vi "SC Deploy Command.vi"(6 "deploying?":bool=TRUE, 7 "close project first?":bool, 8 "error in (no error)":errorcluster, 9 "arguments":string[](array[string]), 10 "title":string, 11 "OK message":string="Done.") -> (0 "error out":errorcluster, 1 "result":string)   [LabVIEW 2023]
doc: "Runs a systemcore-deploy deploy, redeploy or fetch command. When the robot runs a version the project doesn't have (DIVERGED), shows SC Choose Version and runs it again with --resolve; when only the robot has changes (BEHIND), takes them without asking; when the robot's SSH host key changed, asks and runs it again with --trust-new-hostkey. Before a choice that changes the project's files (robot, merge), or before running at all when close project first? is set (a command that always changes them, like checkout), it closes the project, and after showing the result it opens it again."
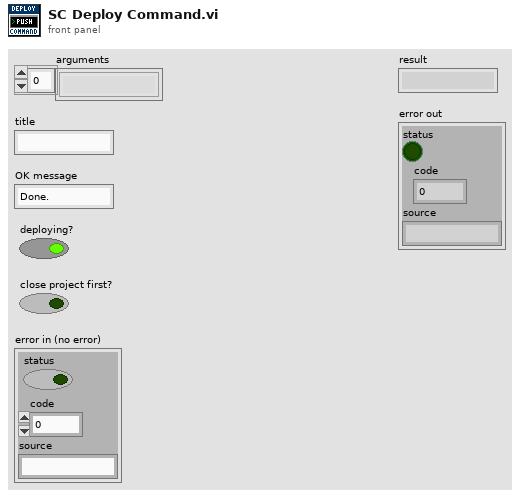
[diagram p1: front panel]
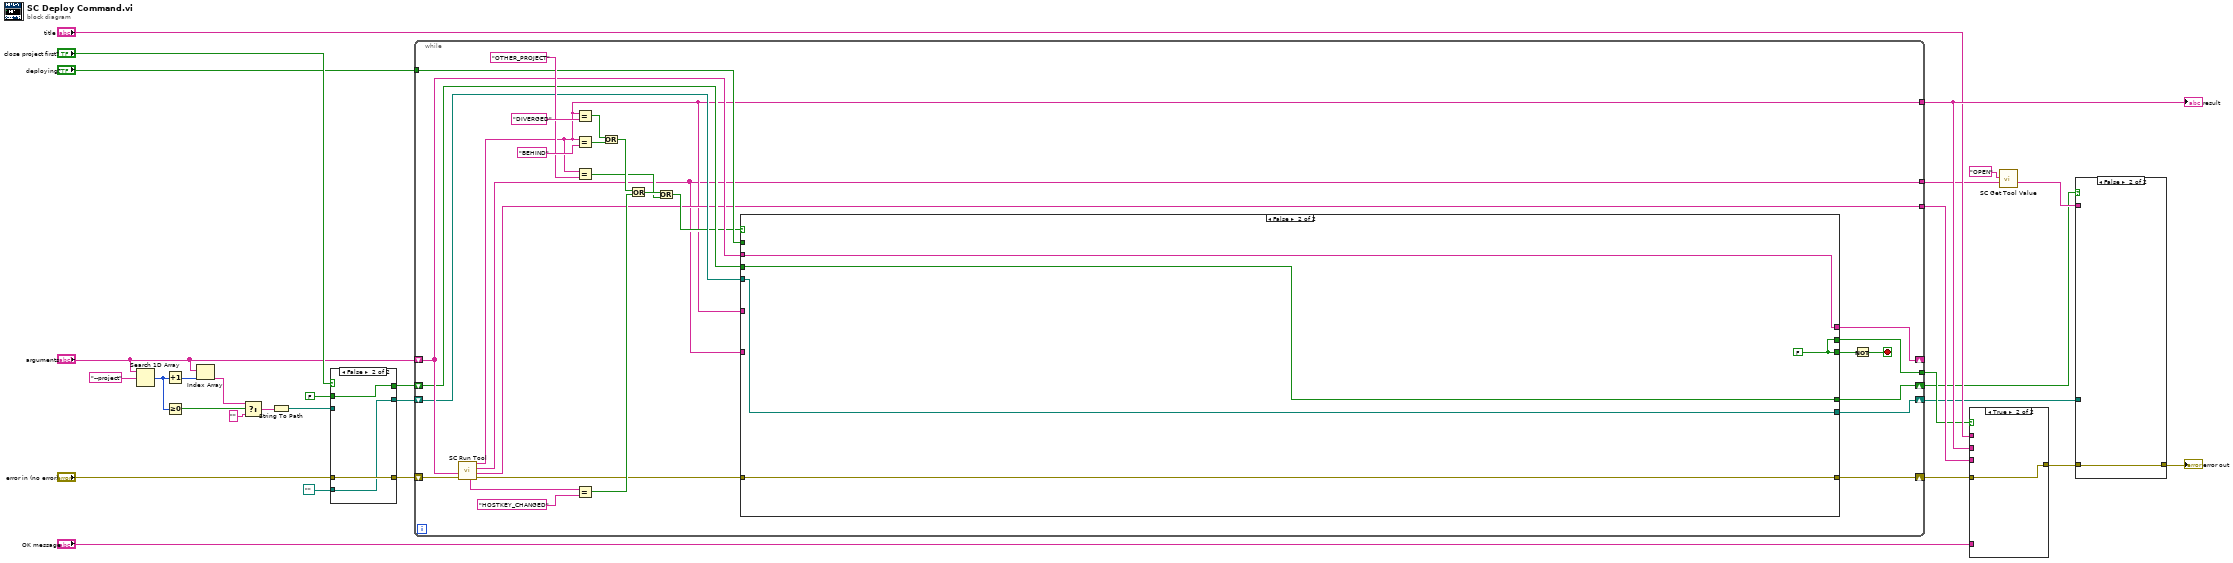
[diagram p0: block diagram]
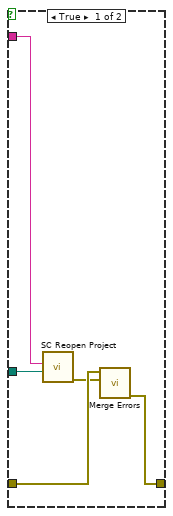
[diagram p2: hidden frame]
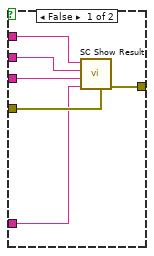
[diagram p3: hidden frame]
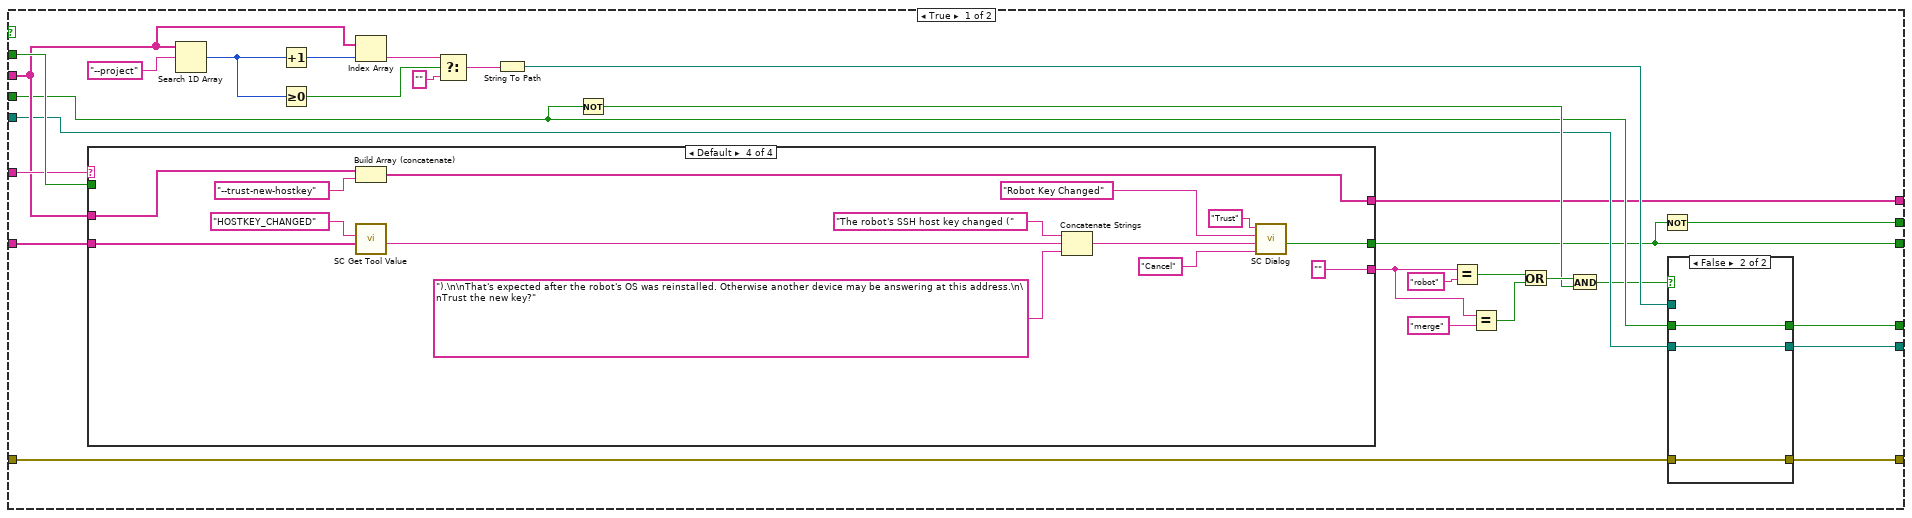
[diagram p4: hidden frame]
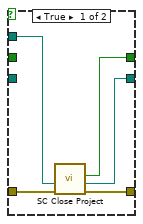
[diagram p5: hidden frame]
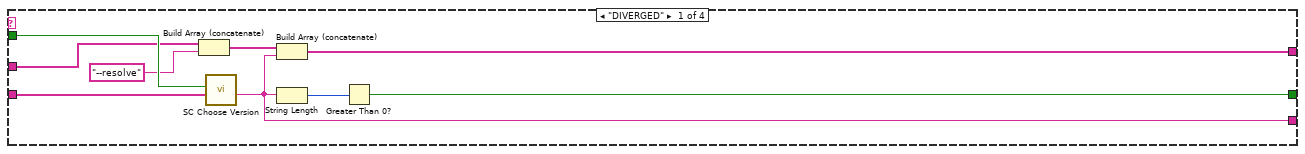
[diagram p6: hidden frame]
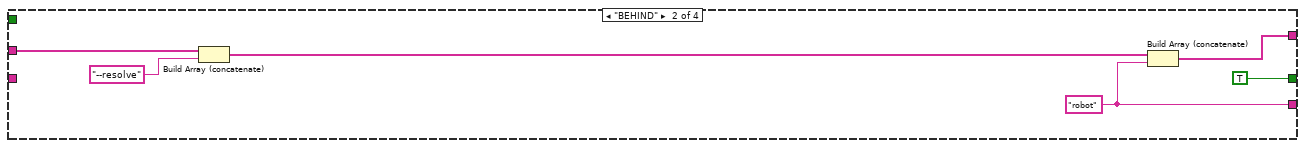
[diagram p7: hidden frame]
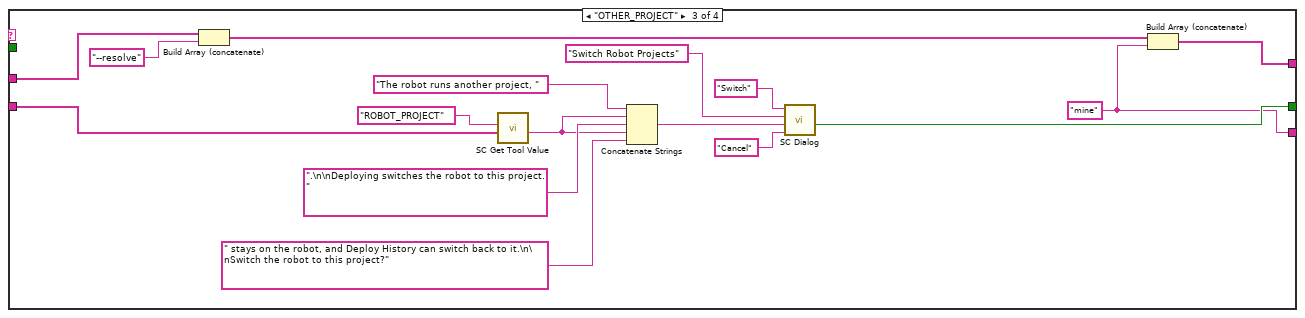
[diagram p8: hidden frame]
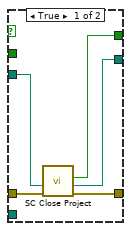
[diagram p9: hidden frame]
diagram:
  n1 = Search 1D Array(1D array="arguments", element="--project") -> (index of element=w28:i32)  [unwired: 1 in]
  n2 = Increment(x=w28) -> (x+1=w29:i32)
  n3 = Greater Or Equal To 0?(x=w28) -> (x >= 0?=w27:bool)
  n4 = Index Array(array="arguments", index=w29) -> (element=w26:string)
  n5 = Select(t=w26, s=w27, f="") -> (s? t:f=w24:string)
  n6 = String To Path(string=w24) -> (path=w20:path)
  n7 = case shown="False" "close project first?" {
    tunnel: "error in (no error)" -> [w35 w38]
    tunnel: FALSE -> [_ w37]
    tunnel: path "" -> [_ w36]
    tunnel: w20 -> [w34 _]
    tunnel: [w33 w38] -> w17
    tunnel: [w32 w37] -> w16
    tunnel: [w31 w36] -> w15
    frame True {
      n8 = call "SC Close Project.vi"("error in (no error)"=w35, "project folder"=w34) -> ("error out"=w33:errorcluster, "project path"=w31:path, "closed?"=w32:bool)  [unwired: 7 in]
    }
    frame False {
    }
  }
  n9 = while {
    shift-right: [w49] -> _
    shift-left: "arguments" -> [w54]
    shift-right: [w48] -> w9
    shift-left: w17 -> [w66]
    shift-right: [w47] -> w1
    shift-left: w16 -> [w51]
    shift-right: [w46] -> w5
    shift-left: w15 -> [w50]
    tunnel: "deploying?" -> [w53]
    tunnel: [w42] -> w13
    tunnel: [w41] -> w12
    tunnel: [w40] -> w8
    tunnel: [w39] -> w7
    stop <- w43 stop-if-true
    n10 = call "SC Run Tool.vi"("error in (no error)"=w66, "arguments"=w54) -> ("error out"=w52:errorcluster, "output"=w42:string, "tool lines"=w39:string[], "result"=w41:string, "result detail"=w63:string)  [unwired: 4 in, 1 out]
    n11 = Equal?(x=w41, y="DIVERGED") -> (x = y?=w61:bool)
    n12 = Equal?(x=w41, y="BEHIND") -> (x = y?=w60:bool)
    n13 = Equal?(x=w41, y="OTHER_PROJECT") -> (x = y?=w55:bool)
    n14 = Equal?(x=w63, y="HOSTKEY_CHANGED") -> (x = y?=w58:bool)
    n15 = Or(x=w61, y=w60) -> (x .or. y?=w59:bool)
    n16 = Or(x=w59, y=w58) -> (x .or. y?=w56:bool)
    n17 = Or(x=w56, y=w55) -> (x .or. y?=w45:bool)
    n18 = case shown="False" w45 {
      tunnel: w54 -> [w84 w153]
      tunnel: w39 -> [w95 _]
      tunnel: w41 -> [w93 _]
      tunnel: w53 -> [w94 _]
      tunnel: w52 -> [w77 w151]
      tunnel: w51 -> [w76 w150]
      tunnel: w50 -> [w75 w149]
      tunnel: [w72 w153] -> w49
      tunnel: [w71 w152] -> w44
      tunnel: [w70 w152] -> w40
      tunnel: [w69 w151] -> w48
      tunnel: [w68 w150] -> w47
      tunnel: [w67 w149] -> w46
      frame True {
        n19 = case shown="Default" w93 {
          tunnel: w84 -> [w109 w118 w124 w139]
          tunnel: w95 -> [w112 _ w134 w148]
          tunnel: w94 -> [w111 _ _ _]
          tunnel: [w106 w115 w121 w137] -> w72
          tunnel: [w105 TRUE w120 w136] -> w71
          tunnel: [w104 w113 w119 ""] -> w91
          frame "DIVERGED" {
            n20 = Build Array (concatenate)(w109, "--resolve") -> (w107:string[])
            n21 = call "SC Choose Version.vi"("tool lines"=w112, "deploying?"=w111) -> ("choice"=w104:string)  [unwired: 9 in]
            n22 = Build Array (concatenate)(w107, w104) -> (w106:string[])
            n23 = String Length(string=w104) -> (length=w110:i32)
            n24 = Greater Than 0?(x=w110) -> (x > 0?=w105:bool)
          }
          frame "BEHIND" {
            w113 = "robot"
            n25 = Build Array (concatenate)(w118, "--resolve") -> (w116:string[])
            n26 = Build Array (concatenate)(w116, w113) -> (w115:string[])
          }
          frame "OTHER_PROJECT" {
            w119 = "mine"
            n27 = Build Array (concatenate)(w124, "--resolve") -> (w122:string[])
            n28 = call "SC Get Tool Value.vi"("tool lines"=w134, "key"="ROBOT_PROJECT") -> ("value"=w130:string)  [unwired: 8 in, 1 out]
            n29 = Concatenate Strings("The robot runs another project, ", w130, ".\n\nDeploying switches the robot to this project. ", w130, " stays on the robot, and Deploy History can switch back to it.\n\nSwitch the robot to this project?") -> (w128:string)
            n30 = call "SC Dialog.vi"("Cancel text"="Cancel", "message"=w128, "window title"="Switch Robot Projects", "OK text"="Switch") -> ("OK?"=w120:bool)  [unwired: 7 in]
            n31 = Build Array (concatenate)(w122, w119) -> (w121:string[])
          }
          frame Default {
            n32 = Build Array (concatenate)(w139, "--trust-new-hostkey") -> (w137:string[])
            n33 = call "SC Get Tool Value.vi"("tool lines"=w148, "key"="HOSTKEY_CHANGED") -> ("value"=w145:string)  [unwired: 8 in, 1 out]
            n34 = Concatenate Strings("The robot's SSH host key changed (", w145, ").\n\nThat's expected after the robot's OS was reinstalled. Otherwise another device may be answering at this address.\n\nTrust the new key?") -> (w143:string)
            n35 = call "SC Dialog.vi"("Cancel text"="Cancel", "message"=w143, "window title"="Robot Key Changed", "OK text"="Trust") -> ("OK?"=w136:bool)  [unwired: 7 in]
          }
        }
        n36 = Search 1D Array(1D array=w84, element="--project") -> (index of element=w82:i32)  [unwired: 1 in]
        n37 = Increment(x=w82) -> (x+1=w83:i32)
        n38 = Greater Or Equal To 0?(x=w82) -> (x >= 0?=w81:bool)
        n39 = Index Array(array=w84, index=w83) -> (element=w80:string)
        n40 = Select(t=w80, s=w81, f="") -> (s? t:f=w78:string)
        n41 = String To Path(string=w78) -> (path=w74:path)
        n42 = Not(x=w76) -> (.not. x?=w86:bool)
        n43 = Equal?(x=w91, y="robot") -> (x = y?=w89:bool)
        n44 = Equal?(x=w91, y="merge") -> (x = y?=w88:bool)
        n45 = Or(x=w89, y=w88) -> (x .or. y?=w87:bool)
        n46 = And(x=w87, y=w86) -> (x .and. y?=w73:bool)
        n47 = Not(x=w71) -> (.not. x?=w70:bool)
        n48 = case shown="False" w73 {
          tunnel: w77 -> [w100 w103]
          tunnel: w76 -> [_ w102]
          tunnel: w75 -> [_ w101]
          tunnel: w74 -> [w99 _]
          tunnel: [w98 w103] -> w69
          tunnel: [w97 w102] -> w68
          tunnel: [w96 w101] -> w67
          frame True {
            n49 = call "SC Close Project.vi"("error in (no error)"=w100, "project folder"=w99) -> ("error out"=w98:errorcluster, "project path"=w96:path, "closed?"=w97:bool)  [unwired: 7 in]
          }
          frame False {
          }
        }
      }
      frame False {
        w152 = FALSE
      }
    }
    n50 = Not(x=w44) -> (.not. x?=w43:bool)
  }
  "result" <- w12
  n51 = case shown="True" w8 {
    tunnel: w13 -> [w158 _]
    tunnel: w12 -> [w157 _]
    tunnel: "title" -> [w156 _]
    tunnel: "OK message" -> [w155 _]
    tunnel: w9 -> [w159 w160]
    tunnel: [w154 w160] -> w3
    frame False {
      n52 = call "SC Show Result.vi"("error in (no error)"=w159, "OK message"=w155, "output"=w158, "result"=w157, "title"=w156) -> ("error out"=w154:errorcluster)  [unwired: 6 in]
    }
    frame True {
    }
  }
  n53 = call "SC Get Tool Value.vi"("tool lines"=w7, "key"="OPEN") -> ("value"=w4:string)  [unwired: 8 in, 1 out]
  n54 = case shown="False" w1 {
    tunnel: w5 -> [w165 _]
    tunnel: w4 -> [w164 _]
    tunnel: w3 -> [w163 w166]
    tunnel: [w161 w166] -> w2
    frame True {
      n55 = call "SC Reopen Project.vi"("project path"=w165, "new file"=w164) -> ("error out"=w162:errorcluster)  [unwired: 9 in]
      n56 = call <vilib>:"Merge Errors.vi"("error in 2 (no error)"=w162, "error in 1 (no error)"=w163) -> ("error out"=w161:errorcluster)  [unwired: 5 in]
    }
    frame False {
    }
  }
  "error out" <- w2
